vi "Get Connector Pane Details.vi"(8 "error in (no error)":errorcluster, 11 "Connector Pane In":refnum<vi>) -> (0 "error out":errorcluster, 2 "Con Pane Details":T1[](array[typedef]), 3 "Connector Pane Out":refnum<vi>)   [LabVIEW 2012, in "Scripting Tools.lvlib"]
uses:
  Scripting Tools.lvlib
  Con Pane Terminal Detail.ctl
  <vilib>/Utility/miscctls.llb/LVRectTypeDef.ctl
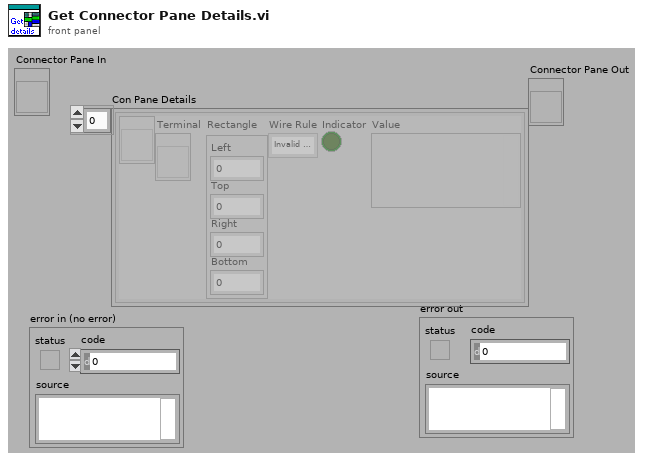
[diagram p1: front panel]
types:
  T1 = typedef "Scripting Tools.lvlib/Con Pane Terminal Detail.ctl" = cluster{"Control":refnum<vi>, "Terminal":refnum<vi>, "Rectangle":T2, "Wire Rule":enum16{"Invalid Wire Rule", "Required", "Recommended", "Optional", "Dynamic Dispatch"}, "Indicator":bool, "Value":variant}
  T2 = typedef "LVRectTypeDef.ctl" = cluster{"Left":i16, "Top":i16, "Right":i16, "Bottom":i16}
  T3 = enum16{"Invalid Wire Rule", "Required", "Recommended", "Optional", "Dynamic Dispatch"}[]
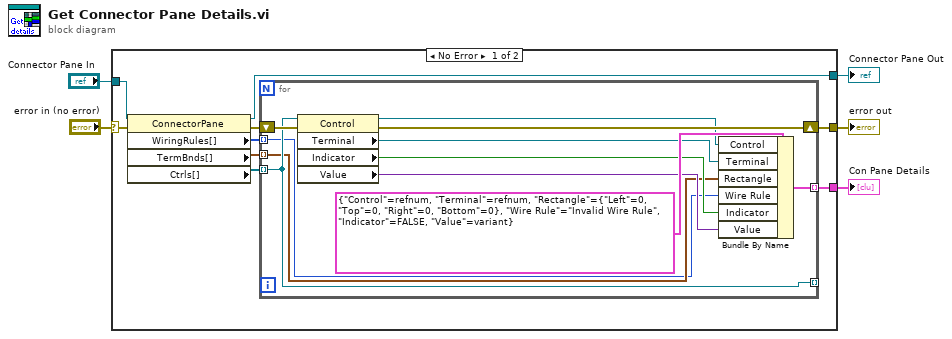
[diagram p0: block diagram]
diagram:
  n1 = case shown="No Error" "error in (no error)" {
    selector: "error in (no error)" -> [w11 w26]
    tunnel: "Connector Pane In" -> [w12 _]
    tunnel: [w14 w26] -> w4
    tunnel: [w13 _] -> w1
    tunnel: [w6 _] -> w5
    frame No Error {
      n2 = property class="ConnectorPane"(reference=w12, error in=w11) -> (reference out=w6:refnum<vi>, error out=w10:errorcluster, "WiringRules[]"=w7:T3, "TermBnds[]"=w8:T2[], "Ctrls[]"=w9:refnum<vi>[])
      n3 = for {
        shift-right: [w24] -> w14
        shift-left: w10 -> [w25]
        tunnel: [w22] -> _ mode=indexing
        tunnel: [w23] -> w13 mode=indexing
        tunnel: w9 -> [w22] mode=indexing
        tunnel: w8 -> [w16] mode=indexing
        tunnel: w7 -> [w15] mode=indexing
        n4 = property class="Control"(reference=w22, error in=w25) -> (reference out=w20:refnum<vi>, error out=w24:errorcluster, "Terminal"=w19:refnum<vi>, "Indicator"=w17:bool, "Value"=w18:variant)
        n5 = Bundle By Name(cluster=T1 {"Control"=refnum, "Terminal"=refnum, "Rectangle"={"Left"=0, "Top"=0, "Right"=0, "Bottom"=0}, "Wire Rule"=enum."Invalid Wire Rule", "Indicator"=FALSE, "Value"=variant} ("Con Pane Terminal Detail"), "Control"=w20, "Terminal"=w19, "Rectangle"=w16, "Wire Rule"=w15, "Indicator"=w17, "Value"=w18) -> (w23:T1)
      }
    }
    frame Error {
    }
  }
  "Connector Pane Out" <- w5
  "error out" <- w4
  "Con Pane Details" <- w1
